vi "Wire XNode Terms by Tag.vi"(7 "TagName":string="phygbuTag", 8 "error in (no error)":errorcluster, 10 "Term Refs":T1[](array[typedef]), 11 "Source References":refnum<vi>[](array[refnum])) -> (0 "error out":errorcluster)   [LabVIEW 2012, in "Scripting Tools.lvlib"]
doc: "Wire as many of the Source references to the TermRefs array as possible based on the Source references being tagged with a string corresponding to the Id of the TermRefs. This is partiocularly useful for wiring up XNodes."
uses:
  Scripting Tools.lvlib
  <vilib>/XNodeSupport/XNodeTermIDPair.ctl
  <vilib>/XNodeSupport/XNodeTermRef.ctl
  <vilib>/XNodeSupport/XNodeString.ctl
  <vilib>/XNodeSupport/NI_XNodeSupport.lvlib
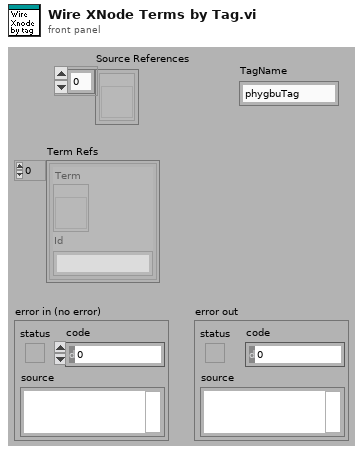
[diagram p1: front panel]
types:
  T1 = typedef "NI_XNodeSupport.lvlib/XNodeTermIDPair.ctl" = cluster{"Term":T2, "Id":T3}
  T2 = typedef "NI_XNodeSupport.lvlib/XNodeTermRef.ctl" = refnum<vi>
  T3 = typedef "NI_XNodeSupport.lvlib/XNodeString.ctl" = string
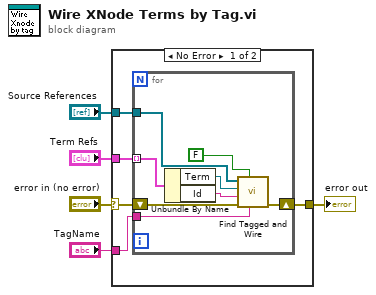
[diagram p0: block diagram]
diagram:
  n1 = case shown="No Error" "error in (no error)" {
    selector: "error in (no error)" -> [w6 w19]
    tunnel: "Source References" -> [w10 _]
    tunnel: "Term Refs" -> [w9 _]
    tunnel: [w8 w19] -> w3
    tunnel: "TagName" -> [w7 _]
    frame No Error {
      n2 = for {
        tunnel: w10 -> [w18]
        tunnel: w9 -> [w17] mode=indexing
        shift-right: [w13] -> w8
        shift-left: w6 -> [w12]
        tunnel: w7 -> [w11]
        n3 = Unbundle By Name(w17) -> ("Term"=w15:T2, "Id"=w16:T3)
        n4 = call "Find Tagged and Wire.vi"("TagName"=w11, "RegExp Search?"=FALSE, "error in (no error)"=w12, "TagValue"=w16, "Single Reference"=w15, "Multiple  References"=w18) -> ("error out"=w13:errorcluster)  [unwired: 5 out]
      }
    }
    frame Error {
    }
  }
  "error out" <- w3
